vi "Edit Scale.vi"(11 "Sacle Setting In":T1) -> (3 "Sacle Setting Out":T1)   [LabVIEW 2020, in "Data Viewer.lvlib" / "Data Viewer.lvclass"]
uses:
  Data Viewer.lvclass
  Scale Setting--cluster.ctl
panel:
  in  "Tab Control":enum32{"Page 2"}(tab)
  in  "对数":bool
  in  "显示网格":bool
  in  "自动标尺":bool
  in  "标尺间隔":dbl format="%.2f"
  in  "标尺最大值":dbl format="%.2f"
  in  "标尺最小值":dbl format="%.2f"
  in  "颜色":u32(colorbox)
  in  "单位":string
  in  "标尺名称":string
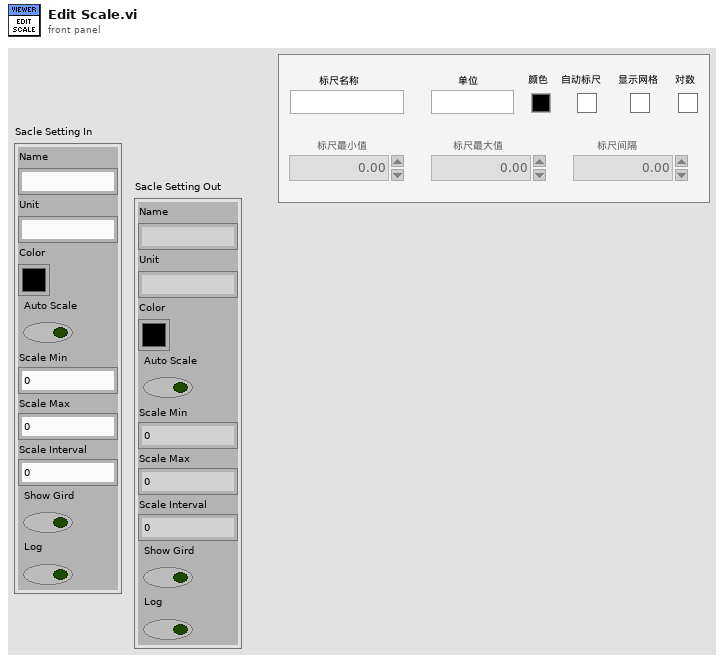
[diagram p1: front panel]
types:
  T1 = typedef "Data Viewer.lvlib/Data Viewer.lvclass/Scale Setting--cluster.ctl" = cluster{"Name":string, "Unit":string, "Color":u32, "Auto Scale":bool, "Scale Min":dbl, "Scale Max":dbl, "Scale Interval":dbl, "Show Gird":bool, "Log":bool}
  T2 = enum32{"Invalid", "Standard", "Closed", "Hidden", "Minimized", "Maximized"}
  T3 = cluster{"初始化":refnum<user-event>, "自动标尺？":refnum<user-event>}
  T4 = enum8{"Enabled", "Disabled", "Disabled and Grayed Out"}
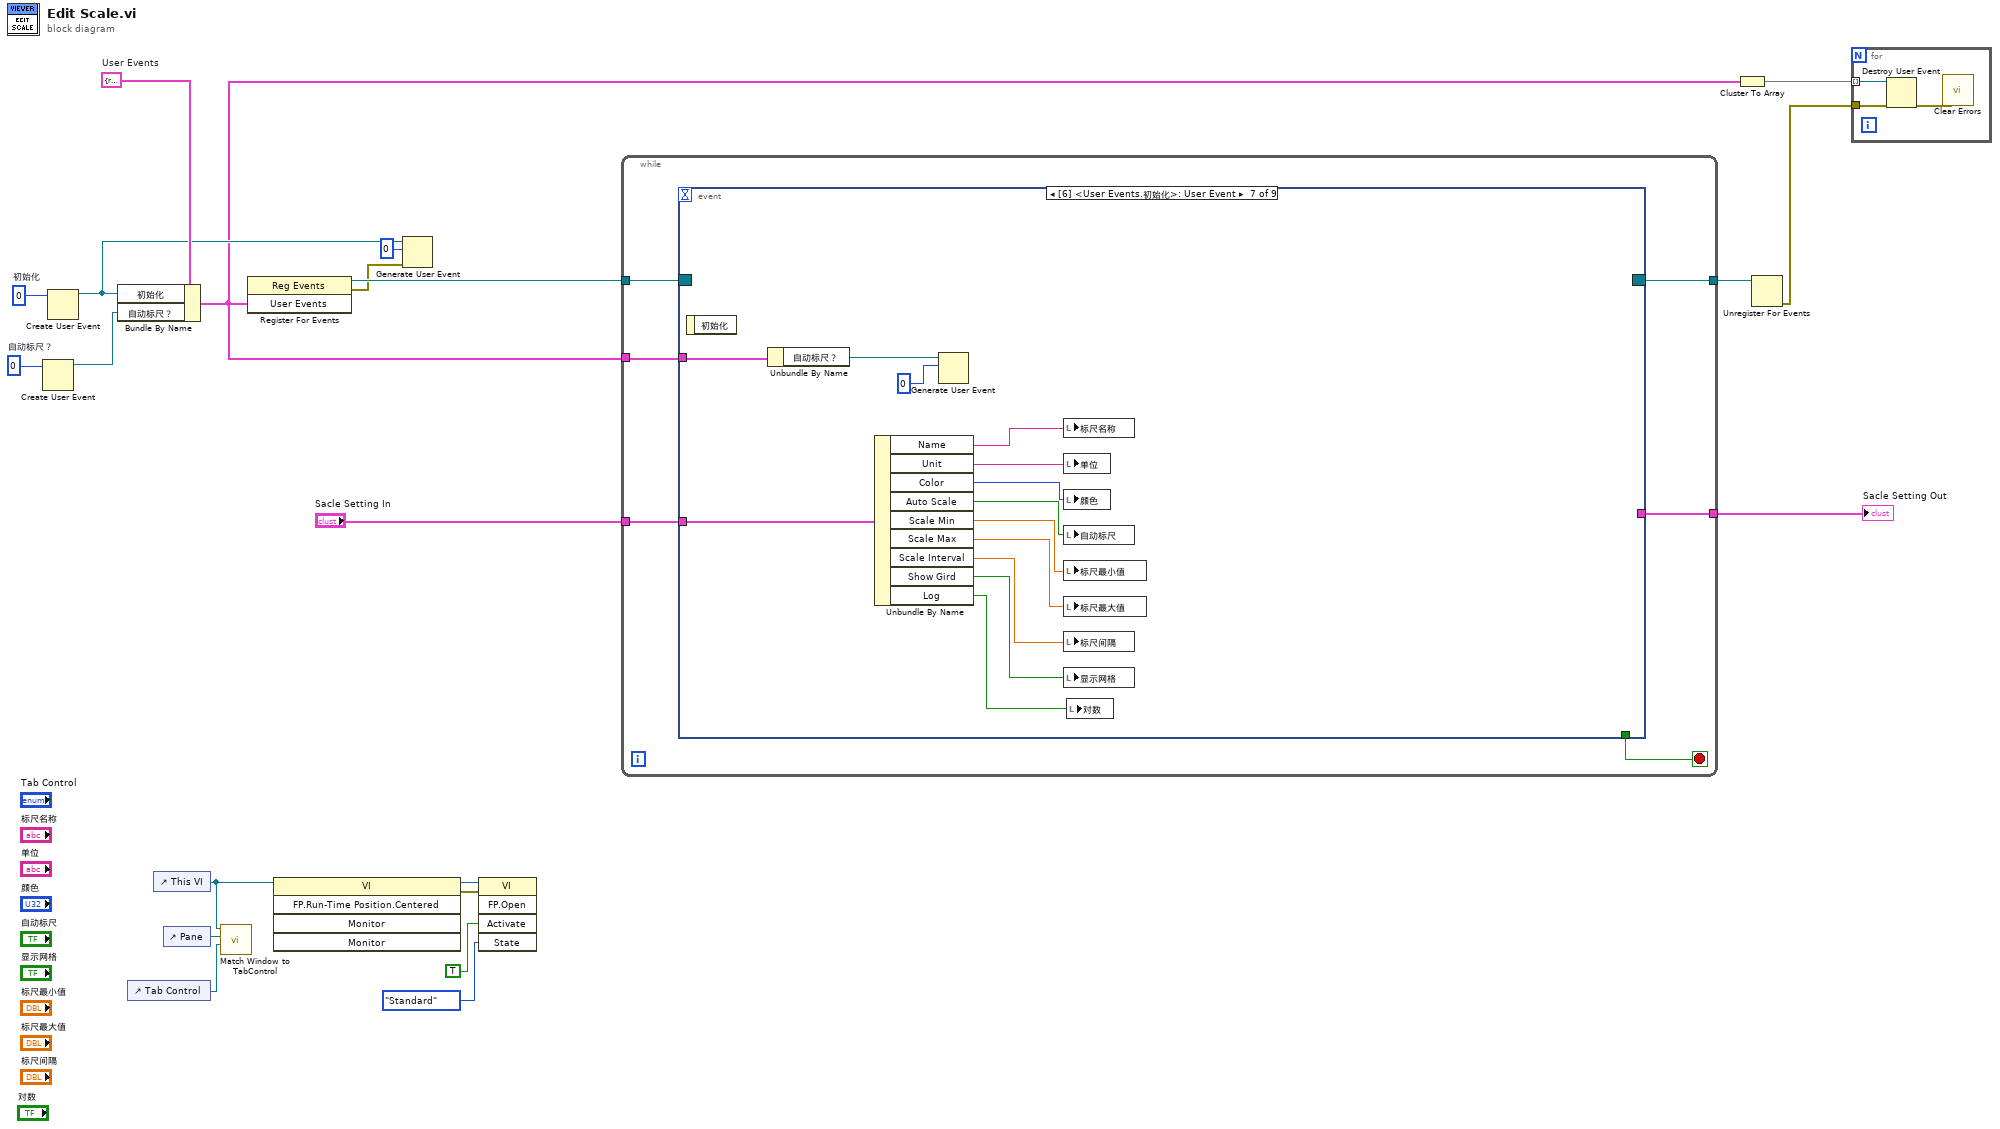
[diagram p0: block diagram]
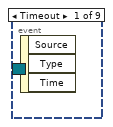
[diagram p2: hidden frame]
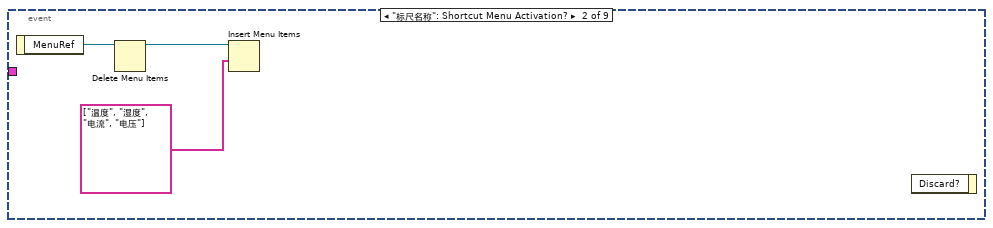
[diagram p3: hidden frame]
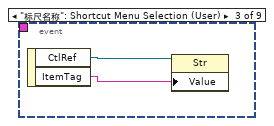
[diagram p4: hidden frame]
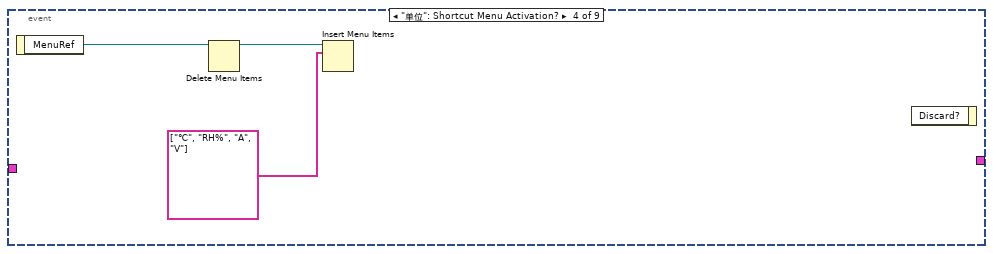
[diagram p5: hidden frame]
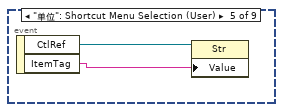
[diagram p6: hidden frame]
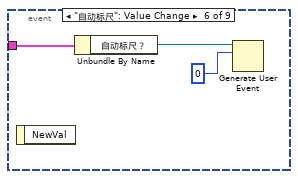
[diagram p7: hidden frame]
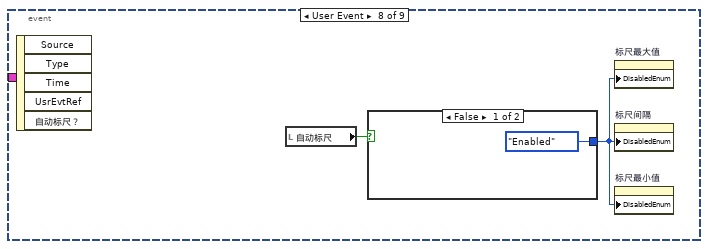
[diagram p8: hidden frame]
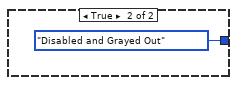
[diagram p9: hidden frame]
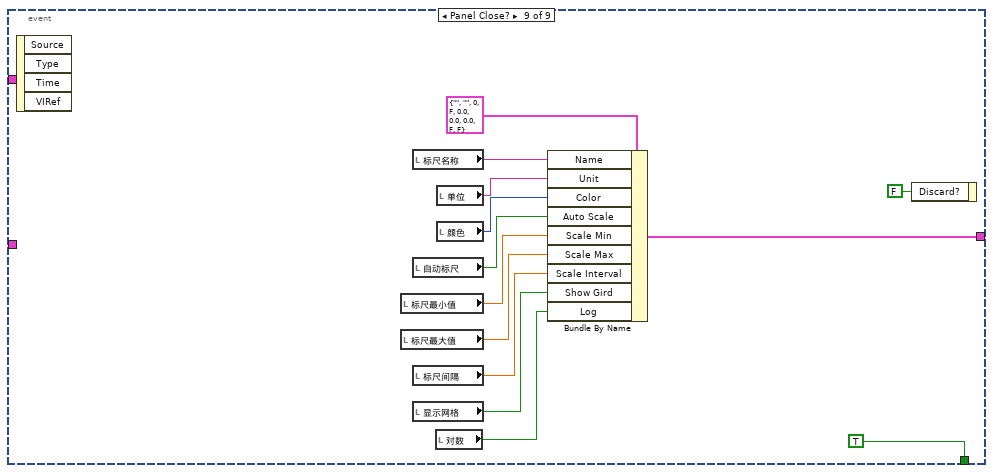
[diagram p10: hidden frame]
diagram:
  w3 = 0  # 自动标尺？
  w18 = T3 {"初始化"=refnum, "自动标尺？"=refnum}  # User Events
  w19 = 0  # 初始化
  n1 = Create User Event(user event datatype=w3) -> (user event=w2:refnum<user-event>)  [unwired: 1 in, 1 out]
  n2 = Create User Event(user event datatype=w19) -> (user event=w16:refnum<user-event>)  [unwired: 1 in, 1 out]
  n3 = Bundle By Name(cluster=w18, "初始化"=w16, "自动标尺？"=w2) -> (w1:T3)
  n4 = control-ref of="Tab Control"() -> (w21:refnum<vi>)
  n5 = control-ref of="This VI"() -> (w13:refnum<vi>)
  n6 = control-ref of="Pane"() -> (w20:refnum<vi>)
  n7 = call "Match Window to TabControl.vi"("Tab Control"=w21, "Pane"=w20, "VI in"=w13) -> ()  [unwired: 9 in]
  n8 = register-events(w1) -> (reference out=w17:refnum<event-registration>, error out=w15:errorcluster)  [unwired: 2 in]
  n9 = invoke class="VI" method="FP.Run-Time Position.Centered"(reference=w13) -> (reference out=w12:refnum<vi>, error out=w11:errorcluster)  [unwired: 4 in, 3 out]
  n10 = Generate User Event(user event=w16, event data cluster=0 ("event data"), error in=w15) -> ()  [unwired: 1 in, 2 out]
  n11 = invoke class="VI" method="FP.Open"(reference=w12, error in=w11, "Activate"=TRUE ("Activate?"), "State"=T2."Standard") -> ()  [unwired: 1 in, 5 out]
  n12 = while {
    tunnel: w17 -> [w26]
    tunnel: "Sacle Setting In" -> [w25]
    tunnel: [w24] -> w7
    tunnel: [w23] -> w4
    tunnel: w1 -> [w22]
    stop <- w27 stop-if-true
    n13 = event shown="[6] <User Events.初始化>: User Event" {
      selector: w26 -> [_ _ _ _ _ _ _ _ _]
      dyn-events: [_ _ _ _ _ _ _ _ _] -> w24
      timeout: _ -> [_ _ _ _ _ _ _ _ _]
      tunnel: [_ _ _ _ _ _ _ _ TRUE] -> w27
      tunnel: w25 -> [_ _ _ _ _ _ w53 _ _]
      tunnel: [_ _ _ _ _ _ _ _ w59] -> w23
      tunnel: w22 -> [_ _ _ _ _ w40 w44 _ _]
      event Timeout {
        n14 = event-data() -> ()  [unwired: 1 in, 3 out]
      }
      event "标尺名称": Shortcut Menu Activation? {
        n15 = event-data() -> ("MenuRef"=w30:refnum<k9>)  [unwired: 1 in]
        n16 = Delete Menu Items(9:w30) -> (3:w29:refnum<k9>)  [unwired: 3 in, 1 out]
        n17 = Insert Menu Items(7:string[] ["温度", "湿度", "电流", "电压"] ("Strings []"), 9:w29) -> ()  [unwired: 4 in, 3 out]
        n18 = event-data() -> ()  [unwired: 2 in, 1 out]
      }
      event "标尺名称": Shortcut Menu Selection (User) {
        n19 = event-data() -> ("CtlRef"=w32:refnum<vi>, "ItemTag"=w31:string)  [unwired: 1 in]
        n20 = property class="Str"(reference=w32, "Value"=w31) -> ()  [unwired: 1 in, 2 out]
      }
      event "单位": Shortcut Menu Activation? {
        n21 = event-data() -> ("MenuRef"=w34:refnum<k9>)  [unwired: 1 in]
        n22 = Delete Menu Items(9:w34) -> (3:w35:refnum<k9>)  [unwired: 3 in, 1 out]
        n23 = Insert Menu Items(8:string[] ["℃", "RH%", "A", "V"] ("Strings []"), 9:w35) -> ()  [unwired: 4 in, 3 out]
        n24 = event-data() -> ()  [unwired: 2 in, 1 out]
      }
      event "单位": Shortcut Menu Selection (User) {
        n25 = event-data() -> ("CtlRef"=w37:refnum<vi>, "ItemTag"=w36:string)  [unwired: 1 in]
        n26 = property class="Str"(reference=w37, "Value"=w36) -> ()  [unwired: 1 in, 2 out]
      }
      event "自动标尺": Value Change {
        n27 = event-data() -> ()  [unwired: 1 in, 1 out]
        n28 = Unbundle By Name(w40) -> ("自动标尺？"=w39:refnum<user-event>)
        n29 = Generate User Event(user event=w39, event data cluster=0 ("event data")) -> ()  [unwired: 2 in, 2 out]
      }
      event User Event {
        n30 = event-data() -> ()  [unwired: 1 in, 1 out]
        n31 = Unbundle By Name(w44) -> ("自动标尺？"=w43:refnum<user-event>)
        n32 = Unbundle By Name(w53) -> ("Name"=w52:string, "Unit"=w51:string, "Color"=w50:u32, "Auto Scale"=w49:bool, "Scale Min"=w48:dbl, "Scale Max"=w47:dbl, "Scale Interval"=w46:dbl, "Show Gird"=w45:bool, "Log"=w41:bool)
        n33 = Generate User Event(user event=w43, event data cluster=0 ("event data")) -> ()  [unwired: 2 in, 2 out]
        n34 = local write "标尺名称"(w52) -> ()
        n35 = local write "单位"(w51) -> ()
        n36 = local write "颜色"(w50) -> ()
        n37 = local write "自动标尺"(w49) -> ()
        n38 = local write "标尺最小值"(w48) -> ()
        n39 = local write "标尺最大值"(w47) -> ()
        n40 = local write "标尺间隔"(w46) -> ()
        n41 = local write "显示网格"(w45) -> ()
        n42 = local write "对数"(w41) -> ()
      }
      event User Event {
        n43 = event-data() -> ()  [unwired: 1 in, 5 out]
        n44 = local read "自动标尺"() -> (w55:bool)
        n45 = case shown="False" w55 {
          tunnel: [T4."Enabled" ("Disabled") T4."Disabled and Grayed Out" ("Disabled")] -> w54
          frame False {
          }
          frame True {
          }
        }
        n46 = property on="标尺最大值" class="DigNum (strict)"("DisabledEnum"=w54) -> ()  [unwired: 2 in, 2 out]
        n47 = property on="标尺间隔" class="DigNum (strict)"("DisabledEnum"=w54) -> ()  [unwired: 2 in, 2 out]
        n48 = property on="标尺最小值" class="DigNum (strict)"("DisabledEnum"=w54) -> ()  [unwired: 2 in, 2 out]
      }
      event Panel Close? {
        n49 = event-data() -> ()  [unwired: 1 in, 4 out]
        n50 = local read "标尺最小值"() -> (w63:dbl)
        n51 = local read "标尺最大值"() -> (w62:dbl)
        n52 = local read "标尺名称"() -> (w67:string)
        n53 = local read "自动标尺"() -> (w64:bool)
        n54 = local read "标尺间隔"() -> (w61:dbl)
        n55 = local read "显示网格"() -> (w60:bool)
        n56 = local read "对数"() -> (w58:bool)
        n57 = local read "单位"() -> (w66:string)
        n58 = local read "颜色"() -> (w65:u32)
        n59 = Bundle By Name(cluster=T1 {"Name"="", "Unit"="", "Color"=0, "Auto Scale"=FALSE, "Scale Min"=0.0, "Scale Max"=0.0, "Scale Interval"=0.0, "Show Gird"=FALSE, "Log"=FALSE} ("Sacle Setting In"), "Name"=w67, "Unit"=w66, "Color"=w65, "Auto Scale"=w64, "Scale Min"=w63, "Scale Max"=w62, "Scale Interval"=w61, "Show Gird"=w60, "Log"=w58) -> (w59:T1)
        n60 = event-data("Discard?"=FALSE) -> ()  [unwired: 1 in, 1 out]
      }
    }
  }
  "Sacle Setting Out" <- w4
  n61 = Cluster To Array(cluster=w1) -> (array=w5:refnum<user-event>[])
  n62 = Unregister For Events(event registration refnum=w7) -> (error out=w6:errorcluster)  [unwired: 1 in]
  n63 = for {
    tunnel: w6 -> [w73]
    tunnel: w5 -> [w72] mode=indexing
    n64 = Destroy User Event(user event=w72, error in=w73) -> (error out=w71:errorcluster)
    n65 = call <vilib>:"Clear Errors.vi"("error in (no error)"=w71) -> ()  [unwired: 5 in, 2 out]
  }
